vi "Read prelaunchSettings.vi"(8 "error in (no error)":errorcluster, 11 "ZM-HWM-hardware_manager in":refnum<class "ZM-HWM-hardware_manager.lvclass">) -> (0 "error out":errorcluster, 2 "ZM-HWM-PRELAUNCH_SETTINGS":T1={"hardware"=refnum, "intervalMs"=500}, 3 "ZM-HWM-hardware_manager out":refnum<class "ZM-HWM-hardware_manager.lvclass">)   [LabVIEW 2020, in "ZM-HWM-hardware_manager.lvlib" / "ZM-HWM-hardware_manager.lvclass"]
doc: "Reads one field of this class's private data. Generated by lvai_create_accessors from the class private data control."
uses:
  ZM-HWM-hardware_manager.lvclass
  hardware/ZM-HW-hardware/ZM-HW-hardware/ZM-HW-hardware.lvclass
  ZM-HWM-hardware_manager.lvclass/ZM-HWM-hardware_manager.ctl
  ZM-HWM-PRELAUNCH_SETTINGS.ctl
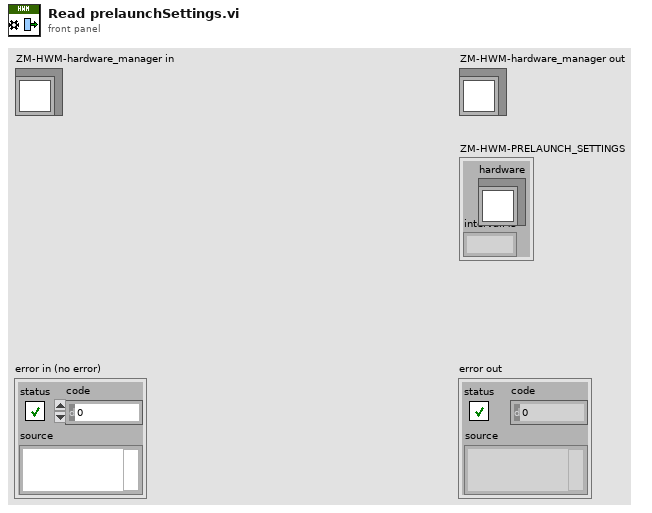
[diagram p1: front panel]
types:
  T1 = typedef "ZM-HWM-hardware_manager.lvlib/ZM-HWM-hardware_manager.lvclass/ZM-HWM-PRELAUNCH_SETTINGS.ctl" = cluster{"hardware":refnum<class "ZM-HW-hardware.lvclass">, "intervalMs":u32}
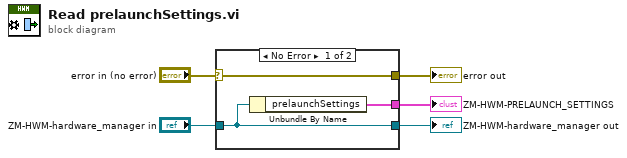
[diagram p0: block diagram]
diagram:
  n1 = case shown="No Error" "error in (no error)" {
    selector: "error in (no error)" -> [w8 w9]
    tunnel: [w8 w9] -> w4
    tunnel: [w7 w10] -> w2
    tunnel: "ZM-HWM-hardware_manager in" -> [w7 w10]
    tunnel: [w6 _] -> w1
    frame No Error {
      n2 = Unbundle By Name(w7) -> ("prelaunchSettings"=w6:T1)
    }
    frame Error {
    }
  }
  "error out" <- w4
  "ZM-HWM-hardware_manager out" <- w2
  "ZM-HWM-PRELAUNCH_SETTINGS" <- w1
